vi "PTestbed_CyclingRT.vi"() -> ()   [LabVIEW 2020]
uses:
  IT-M3400/IT-M3400.lvlib
panel:
  out "end time":u32
  out "initial time":u32
  out "DAQ error out":errorcluster[](array[cluster])
  out "PS error out":errorcluster[](array[cluster])
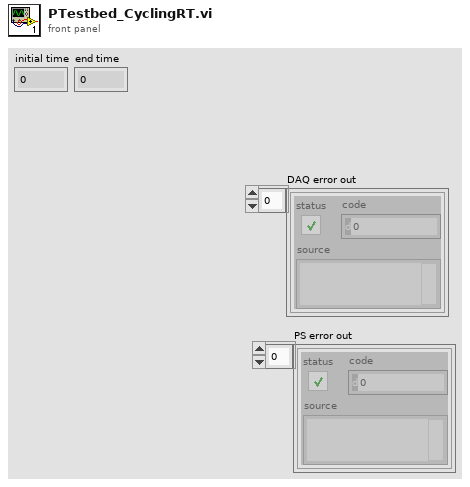
[diagram p1: front panel]
types:
  T1 = enum16{"Battery 1", "Battery 2", "Battery 3", "Battery 1&2", "Battery 1&3", "Battery 2&3", "Battery 1&2&3"}
  T2 = enum16{"\"30Q\"", "\"40T\"", "\"2P30Q\"", "\"3P30Q\"", "\"Nissan Leaf\"", ""}
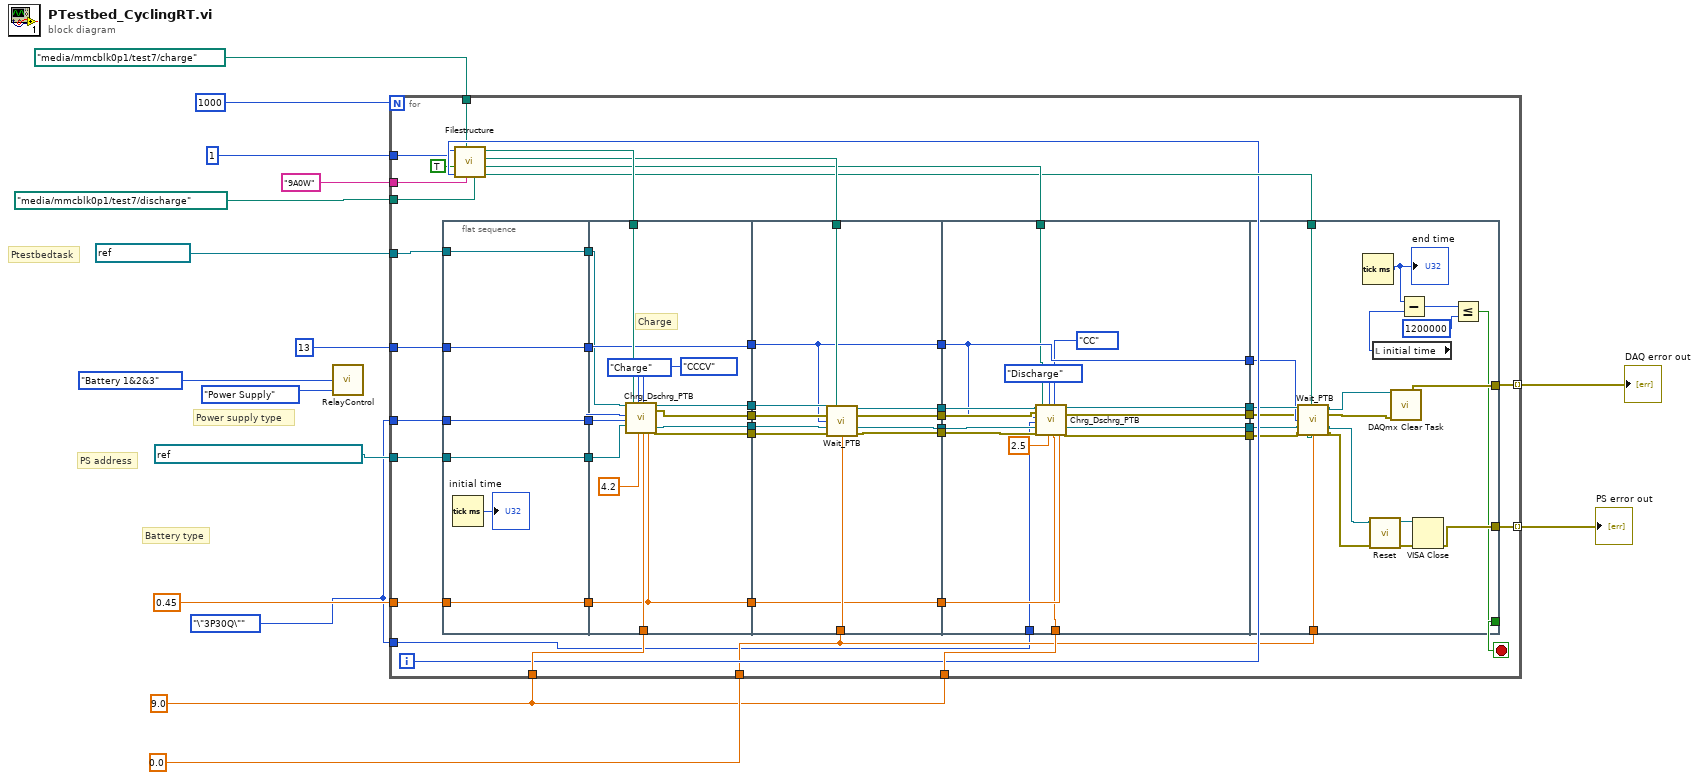
[diagram p0: block diagram]
diagram:
  w3 = 9.0 ("Charge Current Setpoint")
  w1 = T2."\"3P30Q\"" ("Battery Type")
  # "Battery type"
  # "PS address"
  # "Power supply type"
  # "Ptestbedtask"
  n1 = call "RelayControl.vi"("ITECH or Battery Analyzer"=enum16{"Battery Analyzer", "Power Supply"}."Power Supply" ("NHR or Battery Analyzer"), "Battery Select"=T1."Battery 1&2&3") -> ()  [unwired: 3 in]
  n2 = for {
    N: 1000 ("Number of Cycles") -> [_]
    tunnel: 13 ("#DAQ outputs (1-13)") -> [w52]
    tunnel: w3 -> [w51]
    tunnel: w3 -> [w50]
    tunnel: 0.0 ("Wait time") -> [w25]
    tunnel: 1 ("Starting Cycle") -> [w44]
    tunnel: "9A0W" ("Testname") -> [w42]
    tunnel: path "/media/mmcblk0p1/test7/discharge" ("Discharge filepath") -> [w41]
    tunnel: path "/media/mmcblk0p1/test7/charge" ("Charge filepath") -> [w40]
    tunnel: 0.45 ("Current Cutoff") -> [w39]
    tunnel: [w29] -> w8 mode=indexing
    tunnel: [w28] -> w7 mode=indexing
    tunnel: refnum<k21> "PTesbedTask" ("Data Task in") -> [w27]
    tunnel: refnum<visa-resource-name> "TCPIP0::192.168.0.203::inst0::INSTR" ("PS Visa Out") -> [w26]
    tunnel: w1 -> [w24]
    tunnel: w1 -> [w23]
    i -> [w45]
    stop <- w17 stop-if-true
    n3 = flat-sequence {
      tunnel: w24 -> [w62]
      tunnel: w26 -> [w63]
      tunnel: w39 -> [w64]
      tunnel: w52 -> [w65]
      tunnel: w27 -> [w66]
      tunnel: [w66] -> w22
      tunnel: [w65] -> w21
      tunnel: [w64] -> w20
      tunnel: [w63] -> w19
      tunnel: [w62] -> w18
      tunnel: w51 -> [w79]
      tunnel: [w78] -> w60
      tunnel: [w77] -> w59
      tunnel: [w75] -> w58
      tunnel: w49 -> [w76]
      tunnel: [w72] -> w38
      tunnel: [w71] -> w36
      tunnel: [w70] -> w35
      tunnel: w22 -> [w74]
      tunnel: w21 -> [w75]
      tunnel: w20 -> [w72]
      tunnel: w19 -> [w69]
      tunnel: w18 -> [w68]
      tunnel: w60 -> [w92]
      tunnel: w59 -> [w91]
      tunnel: [w90] -> w57
      tunnel: [w89] -> w56
      tunnel: w58 -> [w81]
      tunnel: [w81] -> w55
      tunnel: w48 -> [w88]
      tunnel: w25 -> [w87]
      tunnel: w38 -> [w86]
      tunnel: [w86] -> w37
      tunnel: w36 -> [w85]
      tunnel: w35 -> [w84]
      tunnel: [w83] -> w34
      tunnel: [w82] -> w33
      tunnel: w57 -> [w103]
      tunnel: w56 -> [w102]
      tunnel: w55 -> [w104]
      tunnel: w50 -> [w93]
      tunnel: w47 -> [w97]
      tunnel: [w100] -> w54
      tunnel: [w101] -> w53
      tunnel: w37 -> [w108]
      tunnel: w34 -> [w105]
      tunnel: w33 -> [w106]
      tunnel: [w98] -> w32
      tunnel: [w99] -> w31
      tunnel: [w104] -> w30
      tunnel: w23 -> [w94]
      tunnel: w46 -> [w121]
      tunnel: w54 -> [w125]
      tunnel: w53 -> [w126]
      tunnel: [w128] -> w29
      tunnel: w32 -> [w127]
      tunnel: w31 -> [w123]
      tunnel: [w120] -> w28
      tunnel: w30 -> [w124]
      tunnel: w25 -> [w122]
      tunnel: [w109] -> w17
      frame #0 {
        n4 = Tick Count (ms)() -> (millisecond timer value=→"initial time":u32)
      }
      frame #1 {
        # "Charge"
        n5 = call "Chrg_Dschrg_PTB.vi"("Data Task in"=w74, "#DAQ outputs (1-13)"=w75, "Battery Type"=w68, "PS VISA in 2"=w69, "CyclePath 2"=w76, "Charge/discharge 2"=enum8{"Charge", "Discharge"}."Charge" ("Charge/discharge"), "Charge/Discharge Voltage Setpoint  2"=4.2, "CC or CCCV 2"=enum16{"CC", "CCCV"}."CCCV" ("CC or CCCV"), "Current Setpoint 2"=w79, "Current Cutoff 2"=w72) -> ("data task out"=w71:refnum<k21>, "data task error out"=w70:errorcluster, "PS VISA out"=w78:refnum<visa-resource-name>, "PS error out 2"=w77:errorcluster)  [unwired: 6 in]
      }
      frame #2 {
        n6 = call "Wait_PTB.vi"("Data Task in"=w85, "data task error in"=w84, "#DAQ outputs (1-13)"=w81, "PS VISA in"=w92, "PS error in"=w91, "Wait Filepath"=w88, "Wait time"=w87) -> ("data task out"=w83:refnum<k21>, "data task error out"=w82:errorcluster, "PS Visa Out"=w90:refnum<visa-resource-name>, "PS error out"=w89:errorcluster)  [unwired: 5 in]
      }
      frame #3 {
        n7 = call "Chrg_Dschrg_PTB.vi"("Data Task in"=w105, "data task error in"=w106, "#DAQ outputs (1-13)"=w104, "Battery Type"=w94, "PS VISA in 2"=w103, "PS error in 2"=w102, "CyclePath 2"=w97, "Charge/discharge 2"=enum8{"Charge", "Discharge"}."Discharge" ("Charge/discharge"), "Charge/Discharge Voltage Setpoint  2"=2.5, "CC or CCCV 2"=enum16{"CC", "CCCV"}."CC" ("CC or CCCV"), "Current Setpoint 2"=w93, "Current Cutoff 2"=w108) -> ("data task out"=w98:refnum<k21>, "data task error out"=w99:errorcluster, "PS VISA out"=w100:refnum<visa-resource-name>, "PS error out 2"=w101:errorcluster)  [unwired: 4 in]
      }
      frame #4 {
        n8 = call "Wait_PTB.vi"("Data Task in"=w127, "data task error in"=w123, "#DAQ outputs (1-13)"=w124, "PS VISA in"=w125, "PS error in"=w126, "Wait Filepath"=w121, "Wait time"=w122) -> ("data task out"=w118:refnum<k21>, "data task error out"=w119:errorcluster, "PS Visa Out"=w115:refnum<visa-resource-name>, "PS error out"=w114:errorcluster)  [unwired: 5 in]
        n9 = Tick Count (ms)() -> (millisecond timer value=w113:u32)
        "end time" <- w113
        n10 = call "Reset.vi"("error in"=w114, "VISA resource name"=w115) -> ("error out"=w116:errorcluster, "VISA resource name out"=w117:refnum<visa-resource-name>)  [unwired: 8 in]
        n11 = local read "initial time"() -> (w112:u32)
        n12 = call "DAQmx Clear Task.vi"("task in"=w118, "error in"=w119) -> ("error out"=w120:errorcluster)  [unwired: 13 in]
        n13 = Subtract(x=w113, y=w112) -> (x-y=w111:u32)
        n14 = VISA Close(VISA resource name=w117, error in (no error)=w116) -> (error out=w128:errorcluster)
        n15 = Less Or Equal?(x=w111, y=u32 1200000) -> (x <= y?=w109:bool)
      }
    }
    n16 = call "Filestructure.vi"("Discharge filepath"=w41, "Batteryname"=w42, "Charge filepath"=w40, "For loop i"=w45, "In for loop"=TRUE, "Starting Cycle"=w44) -> ("DischargeWaitPath"=w46:path, "DischargeCyclePath"=w47:path, "ChargeWaitPath"=w48:path, "ChargeCyclePath"=w49:path)  [unwired: 1 in, 1 out]
  }
  "PS error out" <- w8
  "DAQ error out" <- w7
